vi "Ground Station project.vi"() -> ()   [LabVIEW 2020]
uses:
  <vilib>/Instr/_visa.llb/VISA Configure Serial Port (Instr).vi
  <vilib>/Utility/file.llb/Write Delimited Spreadsheet (I64).vi
panel:
  out "Rover Picture":picture
  out "Data Length":u8
  in  "Insert Excel File":path=path "L:/Rover GS/2/Camera Bytes.csv"
  in  "VISA resource name":refnum<visa-resource-name>="COM3"
  out "Stop Scan Response":string
  out "Start Scan Response":string
  out "Capture response":string
  out "Ping Response":string
  out "Front Distance To Obstacle":dbl(knob) scale=0.0..400.0
  out "Gas":dbl(knob) scale=0.0..500.0 scale format="%#_4g"
  out "Front Distance To Obstacle":dbl(knob) scale=0.0..400.0
  out "IR":bool
  out "Humidity":dbl(slide) scale=0.0..100.0
  out "Temperature":dbl(slide) scale=0.0..50.0
  out "SSP Packet":i32[](array[numeric])=[192, 2, 11, 12, 0, 244, 88, 192]
  out "SSP Packet signal":string
  out "Frame Array":i32[](array[numeric])=[2, 11, 12, 0]
  in  "Data Size":string(combo)="0"
  in  "COMMAND":string(combo)="15"
  in  "Destination":string(combo)="1"
  in  "Source":string(combo)="11"
  out "CRC Bytes":u16=22772 format="%.0x"
  in  "WRITE":bool
  out "CRC Received":string
  out "CRC from Calc":string
  out "Num. of incoming bytes":u32
  out "Bytes actually read":u32
  out "Extracted String":string
  out "Frame Validation":string
  in  "READ":bool=TRUE
  out "Message":string
  in  "Delay before Read (ms)":u32=1000
  in  "ByteOrder 2":bool
  in  "ReverseCRC 2":bool
  in  "Polynom 2":u16=4129 format="%.0x"
  out "CRC Value 2":u16=13921 format="%.0x"
  in  "Polynom":u16=4129 format="%.0x"
  in  "ByteOrder":bool
  in  "ReverseCRC":bool
  # "Sending commands"
  # "Receiving Signals"
  # "(in cm)"
  # "Rover Image"
  # "Rover Ground Station\nTeam 5"
  # "Get Telemetry"
  # "Start Flag"
  # "End Flag"
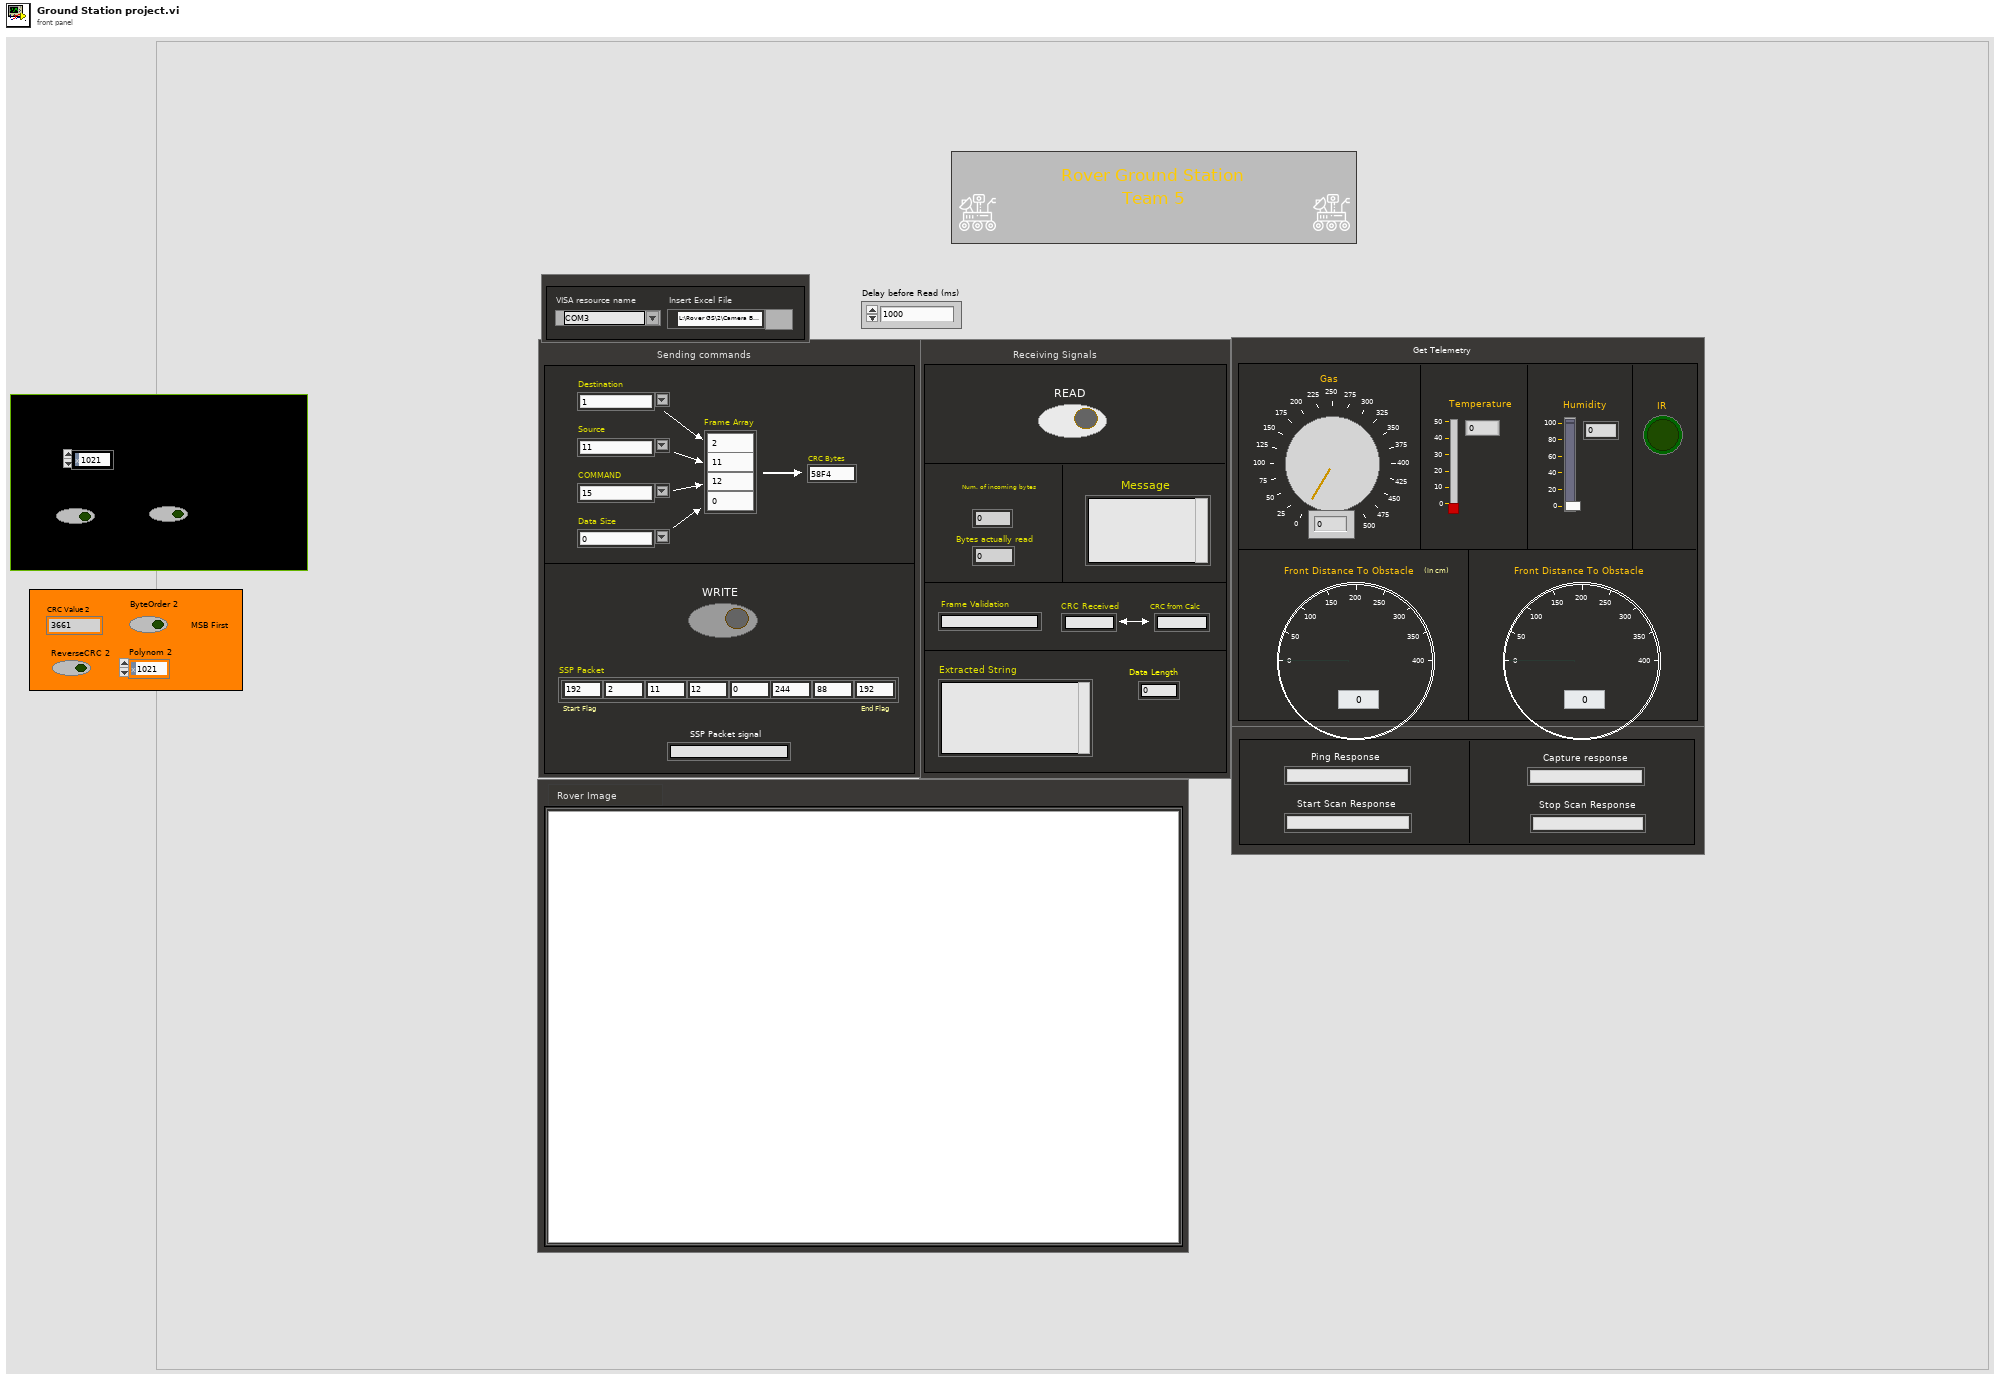
[diagram p1: front panel]
types:
  T1 = typedef "imagedata.ctl" = cluster{"image type":i32, "image depth":i32, "image":u8[], "mask":u8[], "colors":u32[], "Rectangle":cluster{"left":i16, "top":i16, "right":i16, "bottom":i16}}
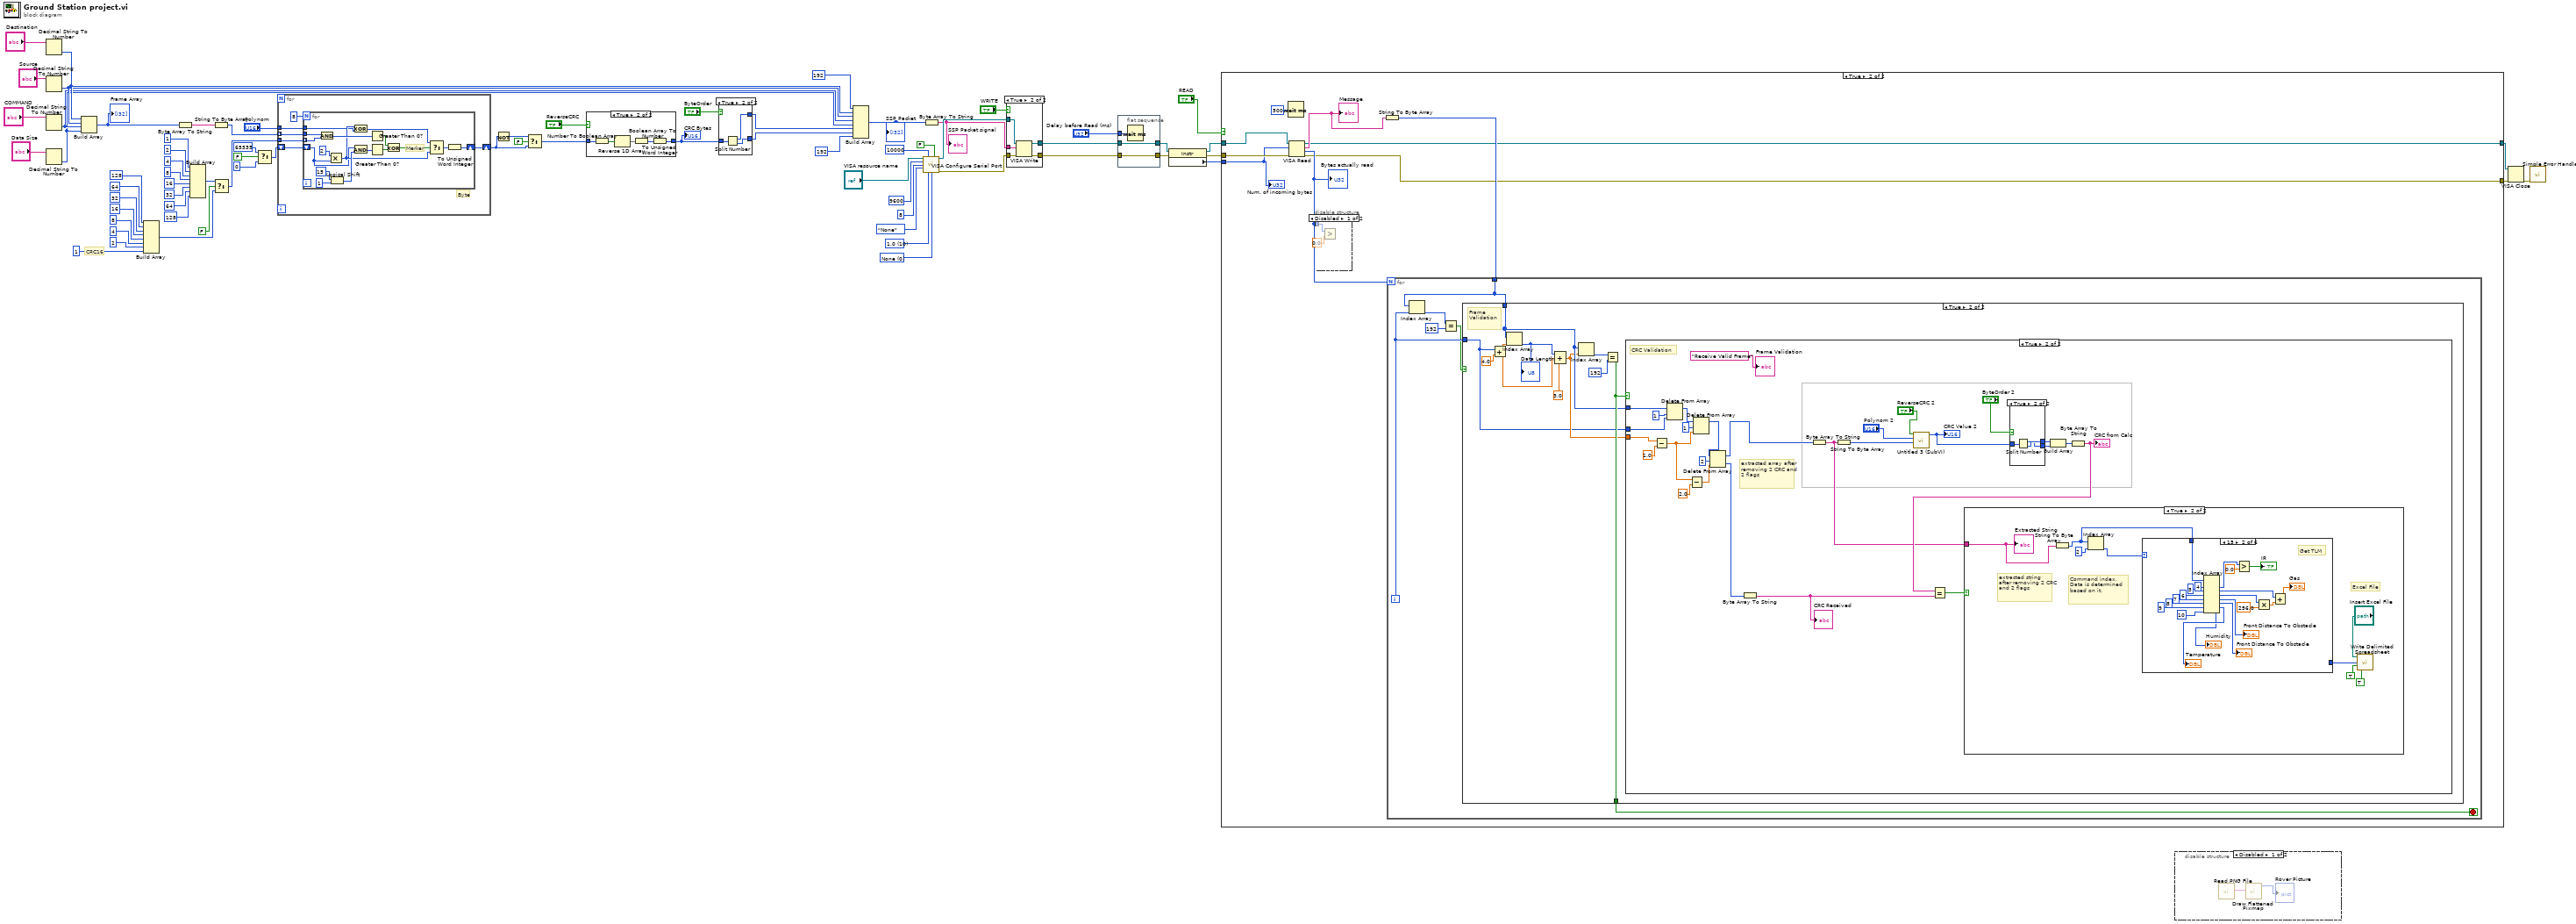
[diagram p0: block diagram]
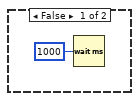
[diagram p2: hidden frame]
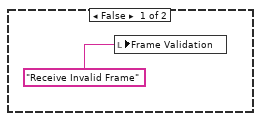
[diagram p5: hidden frame]
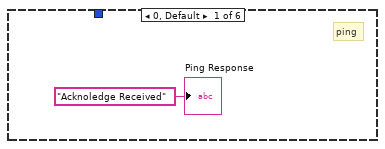
[diagram p7: hidden frame]
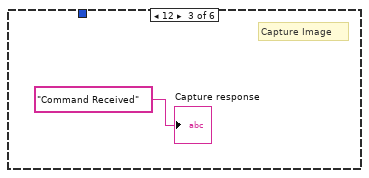
[diagram p8: hidden frame]
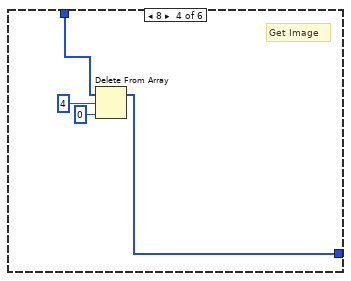
[diagram p9: hidden frame]
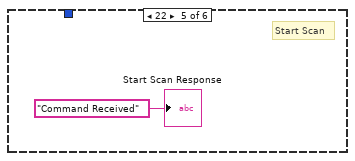
[diagram p10: hidden frame]
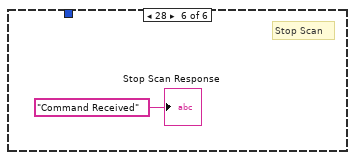
[diagram p11: hidden frame]
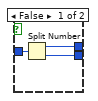
[diagram p12: hidden frame]
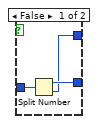
[diagram p15: hidden frame]
diagram:
  w64 = u16 0 items=["None", "XON/XOFF", "RTS/CTS", "XON/XOFF & RTS/CTS", "DTR/DSR", "XON/XOFF & DTR/DSR"] ("flow control (0:none)")
  w65 = u16 10 items=["1.0"=10, "1.5"=15, "2.0"=20] ("stop bits (10: 1 bit)")
  # "CRC16"
  n1 = Decimal String To Number(string="Destination") -> (number=w27:i32)  [unwired: 2 in, 1 out]
  n2 = Decimal String To Number(string="Source") -> (number=w26:i32)  [unwired: 2 in, 1 out]
  n3 = Decimal String To Number(string="COMMAND") -> (number=w25:i32)  [unwired: 2 in, 1 out]
  n4 = Decimal String To Number(string="Data Size") -> (number=w24:i32)  [unwired: 2 in, 1 out]
  n5 = Build Array(w27, w26, w25, w24) -> (w28:i32[])
  "Frame Array" <- w28
  n6 = Build Array(u8 128, u8 64, u8 32, u8 16, u8 8, u8 4, u8 2, u8 1) -> (w44:u8[])
  n7 = Byte Array To String(unsigned byte array=w28) -> (string=w23:string)
  n8 = Build Array(u8 1, u8 2, u8 4, u8 8, u8 16, u8 32, u8 64, u8 128) -> (w43:u8[])
  n9 = String To Byte Array(string=w23) -> (unsigned byte array=w63:u8[])
  n10 = Select(t=w43, s=FALSE, f=w44) -> (s? t:f=w45:u8[])
  n11 = Select(t=u16 65535, s=FALSE, f=u16 0) -> (s? t:f=w62:u16)
  n12 = for {
    shift-right: [w76] -> w40
    shift-left: w62 -> [w78]
    tunnel: w63 -> [w75] mode=indexing
    tunnel: w45 -> [w74]
    tunnel: "Polynom" -> [w73]
    # "Byte"
    n13 = for {
      N: 8 -> [_]
      shift-right: [w94] -> w76
      shift-left: w78 -> [w84]
      tunnel: w74 -> [w85] mode=indexing
      tunnel: w75 -> [w80]
      tunnel: w73 -> [w79]
      # "Merker"
      n14 = And(x=w80, y=w85) -> (x .and. y?=w92:u8)
      n15 = Multiply(x=u16 2, y=w84) -> (x*y=w86:u16)
      n16 = Logical Shift(y=u16 15, x=u16 1) -> (x << y=w88:u16)
      n17 = Exclusive Or(1:w79, 2:w86) -> (0:w95:u16)
      n18 = And(x=w84, y=w88) -> (x .and. y?=w87:u16)
      n19 = Greater Than 0?(x=w92) -> (x > 0?=w91:bool)
      n20 = Greater Than 0?(x=w87) -> (x > 0?=w82:bool)
      n21 = Exclusive Or(1:w82, 2:w91) -> (0:w81:bool)
      n22 = Select(t=w95, s=w81, f=w86) -> (s? t:f=w93:u16)
      n23 = To Unsigned Word Integer(number=w93) -> (unsigned 16bit integer=w94:u16)
    }
  }
  n24 = Not(x=w40) -> (.not. x?=w39:u16)
  n25 = Select(t=w39, s=FALSE, f=w40) -> (s? t:f=w38:u16)
  n26 = case shown="True" "ReverseCRC" {
    tunnel: w38 -> [w96 w101]
    tunnel: [w96 w97] -> w33
    frame False {
    }
    frame True {
      n27 = Number To Boolean Array(number=w101) -> (Boolean array=w100:bool[])
      n28 = Reverse 1D Array(array=w100) -> (reversed array=w99:bool[])
      n29 = Boolean Array To Number(Boolean array=w99) -> (number=w98:u32)
      n30 = To Unsigned Word Integer(number=w98) -> (unsigned 16bit integer=w97:u16)
    }
  }
  "CRC Bytes" <- w33
  n31 = case shown="True" "ByteOrder" {
    tunnel: w33 -> [w104 w107]
    tunnel: [w103 w106] -> w10
    tunnel: [w102 w105] -> w11
    frame False {
      n32 = Split Number(x=w104) -> (hi(x)=w103:u8, lo(x)=w102:u8)
    }
    frame True {
      n33 = Split Number(x=w107) -> (hi(x)=w105:u8, lo(x)=w106:u8)
    }
  }
  n34 = Build Array(192 ("element"), w27, w26, w25, w24, w11, w10, 192 ("element")) -> (w34:i32[])
  "SSP Packet" <- w34
  n35 = call-poly "VISA Configure Serial Port"("VISA resource name"="VISA resource name", "timeout (10sec)"=u32 10000, "Enable Termination\nChar (T)"=FALSE ("Enable Termination\nChar (T)"), "baud rate (9600)"=u32 9600, "data bits (8)"=u16 8, "parity (0:none)"=enum16{"None", "Odd", "Even", "Mark", "Space"}."None", "stop bits (10: 1 bit)"=w65, "flow control (0:none)"=w64) -> ("VISA resource name out"=w72:refnum<visa-resource-name>, "error out"=w71:errorcluster)  [unwired: 6 in]
  n36 = Byte Array To String(unsigned byte array=w34) -> (string=w70:string)
  "SSP Packet signal" <- w70
  n37 = case shown="True" "WRITE" {
    tunnel: [w109 w114] -> w17
    tunnel: [w108 w113] -> w16
    tunnel: w72 -> [w109 w112]
    tunnel: w71 -> [w108 w111]
    tunnel: w70 -> [_ w110]
    frame False {
    }
    frame True {
      n38 = VISA Write(VISA resource name=w112, write buffer=w110, error in (no error)=w111) -> (VISA resource name out=w114:refnum<visa-resource-name>, error out=w113:errorcluster)  [unwired: 1 out]
    }
  }
  n39 = flat-sequence {
    tunnel: w16 -> [w116]
    tunnel: [w116] -> w13
    tunnel: w17 -> [w115]
    tunnel: [w115] -> w15
    tunnel: "Delay before Read (ms)" -> [w117]
    frame #0 {
      n40 = Wait (ms)(milliseconds to wait=w117) -> ()  [unwired: 1 out]
    }
  }
  n41 = property class="Instr"(reference=w15, error in=w13) -> (reference out=w14:refnum<visa-resource-name>, error out=w12:errorcluster, "Serial Settings:Number of Bytes at Serial Port"=w6:u32)
  n42 = case shown="True" "READ" {
    tunnel: w14 -> [_ w127]
    tunnel: w12 -> [_ w126]
    tunnel: w6 -> [_ w124]
    tunnel: [_ w120] -> w3
    tunnel: [_ w119] -> w2
    frame False {
      n43 = Wait (ms)(milliseconds to wait=u32 1000) -> ()  [unwired: 1 out]
    }
    frame True {
      n44 = Wait (ms)(milliseconds to wait=u32 500) -> ()  [unwired: 1 out]
      n45 = VISA Read(VISA resource name=w127, byte count=w124, error in (no error)=w126) -> (VISA resource name out=w120:refnum<visa-resource-name>, read buffer=w121:string, return count=w125:u32, error out=w119:errorcluster)
      "Bytes actually read" <- w125
      "Message" <- w121
      n46 = disable-structure shown="Disabled" {
        disable-tunnel: w125 -> [w129 _]
        frame Disabled {
          n47 = Greater?(x=w129, y=0.0) -> (0:w128:bool)
        }
        frame Enabled {
        }
      }
      n48 = String To Byte Array(string=w121) -> (unsigned byte array=w123:u8[])
      n49 = for {
        N: w125 -> [_]
        tunnel: w123 -> [w134]
        i -> [w133]
        stop <- w131 stop-if-true
        n50 = Index Array(array=w134, index=w133) -> (element=w136:u8)
        n51 = Equal?(x=w136, y=u8 192) -> (x = y?=w132:bool)
        n52 = case shown="True" w132 {
          tunnel: w134 -> [_ w139]
          tunnel: w133 -> [_ w137]
          tunnel: [_ w141] -> w131
          frame False {
          }
          frame True {
            # "Frame Validation"
            n53 = Add(x=w137, y=4.0) -> (x+y=w144:dbl)
            n54 = Index Array(array=w139, index=w144) -> (element=w145:u8)
            "Data Length" <- w145
            n55 = Compound Arithmetic op=ADD(w145, w144, 3.0 ("value")) -> (w138:dbl)
            n56 = Index Array(array=w139, index=w138) -> (element=w142:u8)
            n57 = Equal?(x=w142, y=u8 192) -> (x = y?=w141:bool)
            n58 = case shown="True" w141 {
              tunnel: w139 -> [_ w172]
              tunnel: w138 -> [_ w160]
              tunnel: w137 -> [_ w169]
              frame False {
                n59 = local write "Frame Validation"("Receive Invalid Frame" ("String")) -> ()
              }
              frame True {
                # "CRC Validation"
                # "extracted array after removing 2 CRC and 2 flags"
                n60 = Subtract(x=w160, y=1.0) -> (x-y=w157:dbl)
                n61 = Delete From Array(array=w172, length=1, index=w169) -> (array with subset deleted=w171:u8[])  [unwired: 1 out]
                n62 = Subtract(x=w157, y=2.0) -> (x-y=w156:dbl)
                n63 = Delete From Array(array=w171, length=1, index=w157) -> (array with subset deleted=w155:u8[])  [unwired: 1 out]
                n64 = Delete From Array(array=w155, length=2, index=w156) -> (deleted portion=w154:u8[], array with subset deleted=w153:u8[])
                n65 = Byte Array To String(unsigned byte array=w154) -> (string=w151:string)
                "CRC Received" <- w151
                n66 = Byte Array To String(unsigned byte array=w153) -> (string=w148:string)
                n67 = String To Byte Array(string=w148) -> (unsigned byte array=w168:u8[])
                n68 = call "Untitled 3 (SubVI).vi"("unsigned byte array"=w168, "Polynom"="Polynom 2", "ReverseCRC"="ReverseCRC 2") -> ("CRC Value"=w152:u16)  [unwired: 8 in]
                "CRC Value 2" <- w152
                n69 = case shown="True" "ByteOrder 2" {
                  tunnel: w152 -> [w213 w216]
                  tunnel: [w212 w215] -> w162
                  tunnel: [w211 w214] -> w163
                  frame False {
                    n70 = Split Number(x=w213) -> (hi(x)=w212:u8, lo(x)=w211:u8)
                  }
                  frame True {
                    n71 = Split Number(x=w216) -> (hi(x)=w214:u8, lo(x)=w215:u8)
                  }
                }
                n72 = Build Array(w162, w163) -> (w164:u8[])
                n73 = Byte Array To String(unsigned byte array=w164) -> (string=w150:string)
                "CRC from Calc" <- w150
                n74 = Equal?(x=w150, y=w151) -> (x = y?=w149:bool)
                n75 = case shown="True" w149 {
                  tunnel: w148 -> [_ w182]
                  frame False {
                  }
                  frame True {
                    # "Excel File"
                    # "Command index,\nData is determined based on it."
                    # "extracted string after removing 2 CRC and 2 flags"
                    n76 = String To Byte Array(string=w182) -> (unsigned byte array=w180:u8[])
                    n77 = Index Array(array=w180, index=2) -> (element=w179:u8)
                    n78 = case shown="15" w179 {
                      tunnel: w180 -> [_ w203 _ w206 _ _]
                      tunnel: [_ _ _ w205 _ _] -> w175
                      frame 0, Default {
                        # "ping"
                        "Ping Response" <- "Acknoledge Received"
                      }
                      frame 15 {
                        # "Get TLM"
                        n79 = Index Array(array=w203, index #1=4 ("index"), index #2=5 ("index"), index #3=6 ("index"), index #4=7 ("index"), index #5=8 ("index"), index #6=9 ("index"), index #7=10 ("index")) -> (element #1=w194:u8, element #2=w190:u8, element #3=w191:u8, element #4=→"Front Distance To Obstacle":u8, element #5=→"Front Distance To Obstacle":u8, element #6=→"Temperature":u8, element #7=→"Humidity":u8)
                        n80 = Greater?(x=w194, y=0.0) -> (0:→"IR":bool)
                        n81 = Multiply(x=w191, y=256.0) -> (x*y=w192:dbl)
                        n82 = Add(x=w190, y=w192) -> (x+y=→"Gas":dbl)
                      }
                      frame 12 {
                        # "Capture Image"
                        "Capture response" <- "Command Received"
                      }
                      frame 8 {
                        # "Get Image"
                        n83 = Delete From Array(array=w206, length=4, index=0) -> (array with subset deleted=w205:u8[])  [unwired: 1 out]
                      }
                      frame 22 {
                        # "Start Scan"
                        "Start Scan Response" <- "Command Received"
                      }
                      frame 28 {
                        # "Stop Scan"
                        "Stop Scan Response" <- "Command Received"
                      }
                    }
                    n84 = call-poly <vilib>:"Write Delimited Spreadsheet.vi"("file path (dialog if empty)"="Insert Excel File", "1D data"=w175, "append to file? (new file:F)"=TRUE, "transpose? (no:F)"=TRUE) -> ()  [unwired: 10 in, 2 out]
                    "Extracted String" <- w182
                  }
                }
                "Frame Validation" <- "Receive Valid Frame" ("String")
              }
            }
          }
        }
      }
      "Num. of incoming bytes" <- w124
    }
  }
  n85 = disable-structure shown="Disabled" {
    frame Disabled {
      n86 = call <vilib>:"Read PNG File.vi"() -> ("image data"=w217:T1)  [unwired: 9 in, 2 out]
      n87 = call <vilib>:"Draw Flattened Pixmap.vi"("image data"=w217) -> ("new picture"=→"Rover Picture":picture)  [unwired: 8 in]
    }
    frame Enabled {
    }
  }
  n88 = VISA Close(VISA resource name=w3, error in (no error)=w2) -> (error out=w4:errorcluster)
  n89 = call <vilib>:"Simple Error Handler.vi"("error in (no error)"=w4) -> ()  [unwired: 4 in, 5 out]
